vi "Test_Logic_Caraya.vi"(8 "error in":errorcluster) -> (0 "error out":errorcluster)   [LabVIEW 2026]
doc: "Caraya test of the Logic VIs: Parse Sequence JSON (valid + empty), Lookup Channel (found + missing), Safe Setpoints (zero clamp). Every assert is chained on the error wire after Define Test so that all of them register with the test."
uses:
  <vilib>/addons/_JKI Toolkits/Caraya/classes/Test/Test.lvclass
  <vilib>/addons/_JKI Toolkits/Caraya/classes/Assert/Assert.lvclass
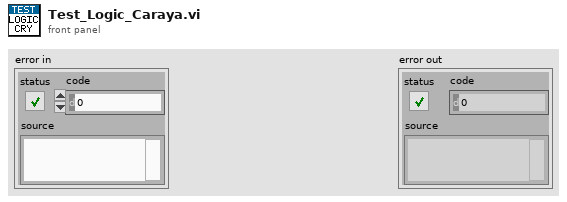
[diagram p1: front panel]
types:
  T1 = cluster{"channels":cluster{"channel":string, "value":dbl}[], "timestamp_ms":dbl}
  T2 = cluster{"rig_id":string, "description":string, "plugin_class":string, "channels":cluster{"name":string, "unit":string, "min":dbl, "max":dbl}[]}
  T3 = typedef "Sequence File.ctl" = cluster{"sequence_id":string, "description":string, "rig_config":string, "steps":T4[]}
  T4 = typedef "Step Config.ctl" = cluster{"step_no":i32, "step_name":string, "command_type":string, "setpoints":T5[], "conditions":T6[], "dwell_time_ms":i32, "timeout_ms":i32, "expected_result":string}
  T5 = typedef "Channel Value.ctl" = cluster{"channel":string, "value":dbl}
  T6 = typedef "Condition.ctl" = cluster{"channel":string, "target":dbl, "tolerance":dbl}
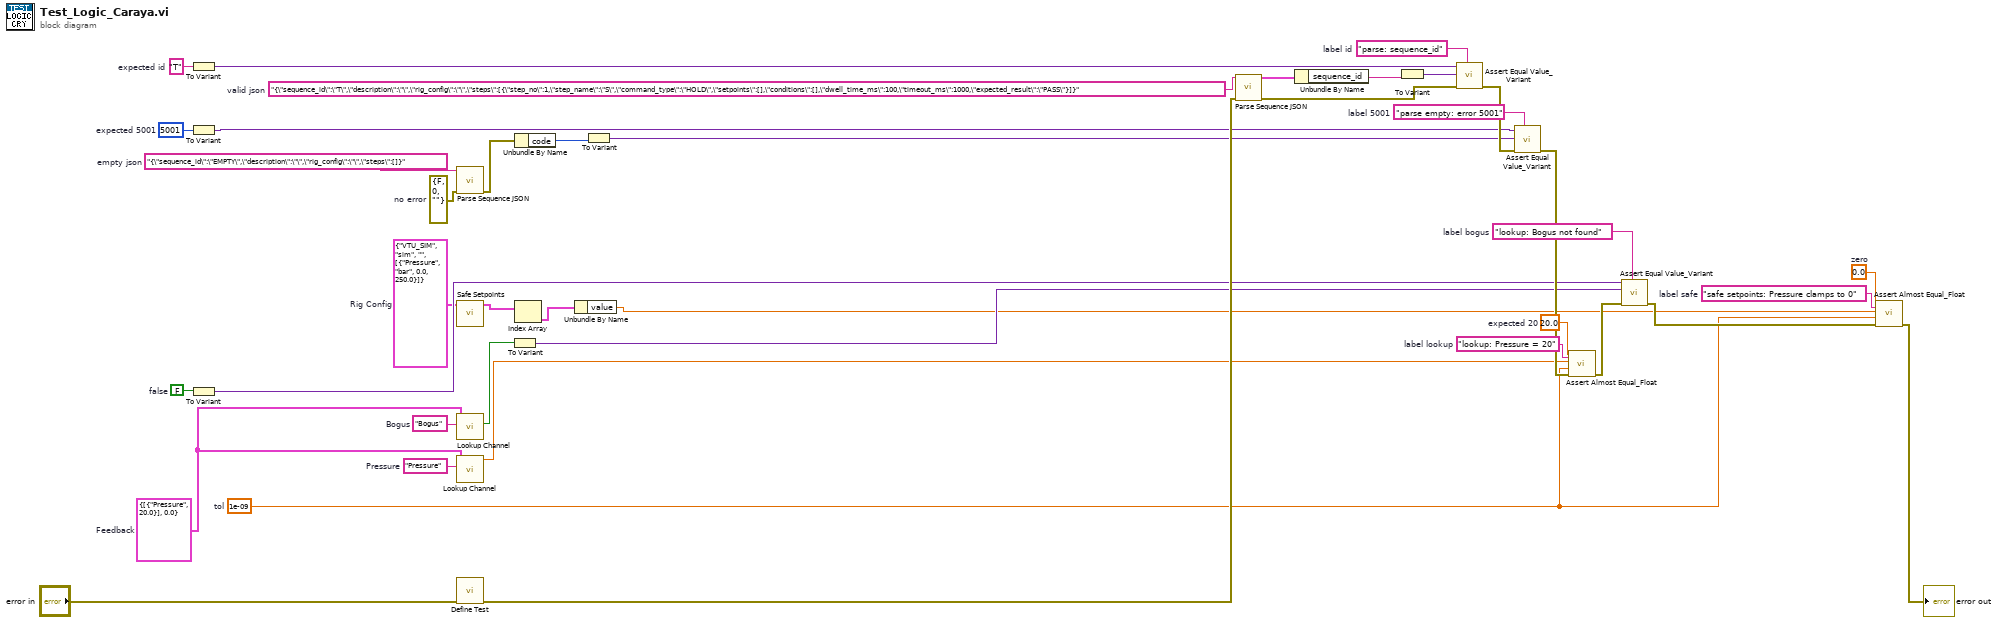
[diagram p0: block diagram]
diagram:
  w6 = "safe setpoints: Pressure clamps to 0"  # label safe
  w2 = 0.0  # zero
  w13 = "lookup: Bogus not found"  # label bogus
  w14 = FALSE  # false
  w21 = "lookup: Pressure = 20"  # label lookup
  w18 = 20.0  # expected 20
  w26 = "parse empty: error 5001"  # label 5001
  w27 = 5001  # expected 5001
  w35 = "parse: sequence_id"  # label id
  w36 = "T"  # expected id
  w4 = 1e-09  # tol
  w30 = errorcluster {"status"=FALSE, "code"=0, "source"=""}  # no error
  w17 = "Bogus"  # Bogus
  w22 = "Pressure"  # Pressure
  w16 = T1 {"channels"=[{"channel"="Pressure", "value"=20.0}], "timestamp_ms"=0.0}  # Feedback
  w9 = T2 {"rig_id"="VTU_SIM", "description"="sim", "plugin_class"="", "channels"=[{"name"="Pressure", "unit"="bar", "min"=0.0, "max"=250.0}]}  # Rig Config
  w31 = "{\"sequence_id\":\"EMPTY\",\"description\":\"\",\"rig_config\":\"\",\"steps\":[]}"  # empty json
  w40 = "{\"sequence_id\":\"T\",\"description\":\"\",\"rig_config\":\"\",\"steps\":[{\"step_no\":1,\"step_name\":\"S\",\"command_type\":\"HOLD\",\"setpoints\":[],\"conditions\":[],\"dwell_time_ms\":100,\"timeout_ms\":1000,\"expected_result\":\"PASS\"}]}"  # valid json
  n1 = To Variant(anything=w36) -> (Variant=w32:variant)
  n2 = To Variant(anything=w27) -> (Variant=w23:variant)
  n3 = To Variant(anything=w14) -> (Variant=w10:variant)
  n4 = call "Parse Sequence JSON.vi"("error in"=w30, "JSON string"=w31) -> ("error out"=w29:errorcluster)  [unwired: 8 in, 1 out]
  n5 = call "Safe Setpoints.vi"("Rig Config"=w9) -> ("setpoints"=w8:cluster{"channel":string, "value":dbl}[])  [unwired: 10 in]
  n6 = call "Lookup Channel.vi"("channel"=w17, "Channel Feedback"=w16) -> ("found"=w15:bool)  [unwired: 8 in, 1 out]
  n7 = call "Lookup Channel.vi"("channel"=w22, "Channel Feedback"=w16) -> ("value"=w19:dbl)  [unwired: 8 in, 1 out]
  n8 = call <vilib>:"Define Test.vi"("error in (no error)"="error in") -> ("error out"=w39:errorcluster)  [unwired: 9 in, 1 out]
  n9 = To Variant(anything=w15) -> (Variant=w11:variant)
  n10 = Unbundle By Name(w29) -> ("code"=w28:i32)
  n11 = Index Array(array=w8) -> (element=w7:cluster{"channel":string, "value":dbl})  [unwired: 1 in]
  n12 = Unbundle By Name(w7) -> ("value"=w3:dbl)
  n13 = To Variant(anything=w28) -> (Variant=w24:variant)
  n14 = call "Parse Sequence JSON.vi"("error in"=w39, "JSON string"=w40) -> ("error out"=w34:errorcluster, "Sequence File"=w38:T3)  [unwired: 8 in]
  n15 = Unbundle By Name(w38) -> ("sequence_id"=w37:string)
  n16 = To Variant(anything=w37) -> (Variant=w33:variant)
  n17 = call <vilib>:"Assert Equal Value_Variant.vi"("Label"=w35, "error in (no error)"=w34, "Actual"=w33, "Expected"=w32) -> ("error out"=w25:errorcluster)  [unwired: 6 in, 1 out]
  n18 = call <vilib>:"Assert Equal Value_Variant.vi"("Label"=w26, "error in (no error)"=w25, "Actual"=w24, "Expected"=w23) -> ("error out"=w20:errorcluster)  [unwired: 6 in, 1 out]
  n19 = call <vilib>:"Assert Almost Equal_Float.vi"("Label"=w21, "error in (no error)"=w20, "Tolerance"=w4, "Actual"=w19, "Expected"=w18) -> ("error out"=w12:errorcluster)  [unwired: 5 in, 1 out]
  n20 = call <vilib>:"Assert Equal Value_Variant.vi"("Label"=w13, "error in (no error)"=w12, "Actual"=w11, "Expected"=w10) -> ("error out"=w5:errorcluster)  [unwired: 6 in, 1 out]
  n21 = call <vilib>:"Assert Almost Equal_Float.vi"("Label"=w6, "error in (no error)"=w5, "Tolerance"=w4, "Actual"=w3, "Expected"=w2) -> ("error out"=→"error out":errorcluster)  [unwired: 5 in, 1 out]
